vi "Write Log.vi"(8 "error in (no error)":errorcluster, 10 "formatted record":string, 11 "handler name":string) -> (0 "error out":errorcluster)   [LabVIEW 2018, in "GLog.lvlib" / "UI Updater.lvlib"]
uses:
  UI Updater.lvlib
  Events/Write Log.ctl
panel:
  # "Connector Pane"
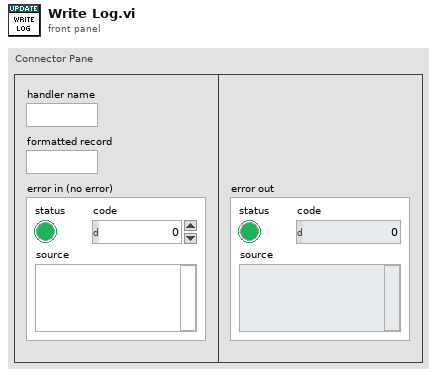
[diagram p1: front panel]
types:
  T1 = typedef "GLog.lvlib/UI Updater.lvlib/Write Log.ctl" = cluster{"handler name":string, "formatted record":string}
  T2 = typedef "GLog.lvlib/UI Updater.lvlib/Events.ctl" = cluster{"Write Log":refnum<user-event>, "Register":refnum<user-event>, "Unregister":refnum<user-event>}
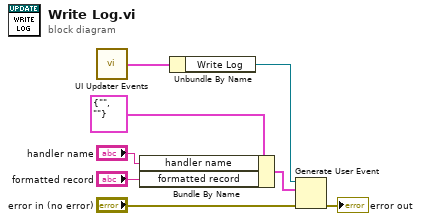
[diagram p0: block diagram]
diagram:
  n1 = call "UI Updater Events.vi"() -> ("UI Updater"=w3:T2)  [unwired: 1 in]
  n2 = Bundle By Name(cluster=T1 {"handler name"="", "formatted record"=""} ("event data"), "handler name"="handler name", "formatted record"="formatted record") -> (w8:T1)
  n3 = Unbundle By Name(w3) -> ("Write Log"=w4:refnum<user-event>)
  n4 = Generate User Event(user event=w4, event data cluster=w8, error in="error in (no error)") -> (error out=→"error out":errorcluster)  [unwired: 1 in, 1 out]
